vi "CalculateSpecificationBuildOrder.vi"(6 "UpdateList":T1, 8 "error in (no error)":errorcluster, 11 "SolutionBuilder in":refnum<class "SolutionBuilder.lvclass">) -> (0 "error out":errorcluster, 3 "SolutionBuilder out":refnum<class "SolutionBuilder.lvclass">)   [LabVIEW 2019, in "SolutionBuilder.lvlib" / "SolutionBuilder.lvclass"]
uses:
  SolutionBuilder.lvclass
  Events/EventUpdateList.ctl
  SolutionBuilder.lvclass/SolutionBuilder.ctl
  SolutionBuilder.lvlib
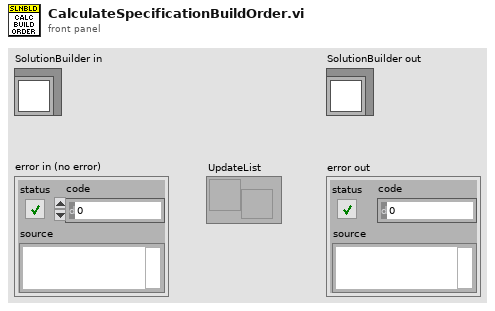
[diagram p1: front panel]
types:
  T1 = typedef "SolutionBuilder.lvlib/EventUpdateList.ctl" = refnum<user-event>
  T2 = typedef "SolutionBuilder.lvlib/SolutionBuilder.lvclass/OrderingMap.ctl" = map{cluster{"Owning project":path, "Build spec name":string, "Target":string}, cluster{"ProjectItem out":refnum<class "ProjectItem.lvclass">, "Deps":set{string}}}
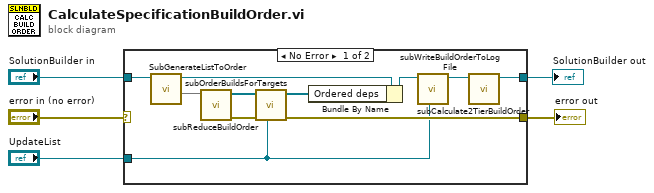
[diagram p0: block diagram]
diagram:
  n1 = case shown="No Error" "error in (no error)" {
    selector: "error in (no error)" -> [_ w18]
    tunnel: "UpdateList" -> [w8 _]
    tunnel: "SolutionBuilder in" -> [w16 w17]
    tunnel: [w7 w17] -> w3
    tunnel: [w9 w18] -> w1
    frame No Error {
      n2 = call "SubGenerateListToOrder.vi"("SolutionBuilder in"=w16) -> ("Ordering map"=w13:T2, "SolutionBuilder out"=w15:refnum<class "SolutionBuilder.lvclass">)  [unwired: 8 in, 1 out]
      n3 = call "subReduceBuildOrder.vi"("Ordering map"=w13) -> ("error out"=w10:errorcluster, "Raw build order"=w12:refnum<class "ProjectItem.lvclass">[])  [unwired: 9 in]
      n4 = call "subOrderBuildsForTargets.vi"("User Event in"=w8, "error in"=w10, "Raw build order in"=w12) -> ("error out"=w9:errorcluster, "Build order"=w11:refnum<class "ProjectItem.lvclass">[])  [unwired: 7 in]
      n5 = Bundle By Name(cluster=w15, "Ordered deps"=w11) -> (w14:refnum<class "SolutionBuilder.lvclass">)
      n6 = call "subCalculate2TierBuildOrder.vi"("UpdateList"=w8, "SolutionBuilder in"=w14) -> ("SolutionBuilder out"=w6:refnum<class "SolutionBuilder.lvclass">)  [unwired: 8 in, 1 out]
      n7 = call "subWriteBuildOrderToLogFile.vi"("SolutionBuilder in"=w6) -> ("SolutionBuilder out"=w7:refnum<class "SolutionBuilder.lvclass">)  [unwired: 9 in, 1 out]
    }
    frame Error {
    }
  }
  "error out" <- w1
  "SolutionBuilder out" <- w3
